vi "AlliGator Clear Parameter & Map Set Rings.vi"(8 "Error In":errorcluster) -> (0 "Error Out":errorcluster)   [LabVIEW 2021, in "AlliGator Parameter Map.lvlib"]
uses:
  AlliGator Parameter Map.lvlib
  AlliGator Parameter Map Control Refnums.ctl
  Globals, Variables, Constants/AlliGator Refnums List.ctl
  GUI/AlliGator GUI.lvlib
panel:
  # "see the License on the block diagram (Ctrl+E or Window:Show Block Diagram)"
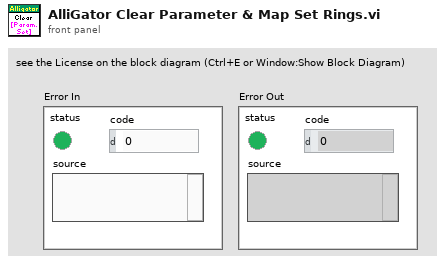
[diagram p1: front panel]
types:
  T1 = typedef "AlliGator GUI.lvlib/AlliGator Refnums List.ctl" = enum16{"---------- AlliGator Control Refnums ----------", "AlliGator Tab Control Refnum", "Dataset Ctrl Refnums", "Image Histogram Ctrl Refnums", "Intensity Time Trace Ctrl Refnums", "Decay Graph Ctrl Refnums", "Decay Statistics Graph Ctrl Refnums", "Phasor Graph Ctrl Refnums", "Phasor Ratio Graph Ctrl Refnums", "Phasor Plot Ctrl Refnums", "Lifetime & Other Parameters Ctrl Refnums", "Decay Fit Parameter Map Ctrl Refnums", "Parameter Map Ctrl Refnums", "Other AlliGator Ctrl Refnums", "---------- AlliGator Menu Refnums ----------", "AlliGator Menu", "---------- AlliGator VI Refnums ----------", "AlliGator Refnum", "AlliGator Settings Refnum", "AlliGator Launcher Refnum", "---------- IO Device ID ----------", "Mouse ID", "Keyboard ID"}
  T2 = typedef "AlliGator Parameter Map.lvlib/AlliGator Parameter Map Control Refnums.ctl" = cluster{"Parameter Map Color Scale":refnum<vi>, "Map Parameter":refnum<vi>, "Max Parameter":refnum<vi>, "Min Parameter":refnum<vi>, "Parameter Map Display":refnum<vi>, "Parameter Map Display Range":refnum<vi>, "Parameter Map Set":refnum<vi>, "Parameter Map X":refnum<vi>, "Parameter Map Y":refnum<vi>, "Parameter Map Value":refnum<vi>}
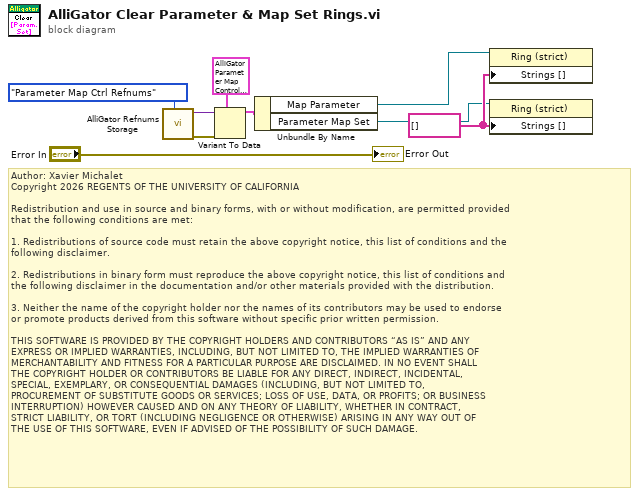
[diagram p0: block diagram]
diagram:
  w8 = string[] [] ("Strings []")
  # "Author: Xavier Michalet\nCopyright 2026 REGENTS OF THE UNIVERSITY OF CALIFORNIA\n\nRedistribution and use in source and binary forms, with or without modification, are permitted provided\nthat the following conditions are met:\n\n1. Redistributions of source code must retain the above copyright notice, this list of conditions and the\nfollowing disclaimer.\n\n2. Redistributions in binary form must reproduce the above copyright notice, this list of conditions and\nthe following disclaimer in the documentation and/or other materials provided with the distribution.\n\n3. Neither the name of the copyright holder nor the names of its contributors may be used to endorse \nor promote products derived from this software without specific prior written permission.\n\nTHIS SOFTWARE IS PROVIDED BY THE COPYRIGHT HOLDERS AND CONTRIBUTORS “AS IS” AND ANY \nEXPRESS OR IMPLIED WARRANTIES, INCLUDING, BUT NOT LIMITED TO, THE IMPLIED WARRANTIES OF\nMERCHANTABILITY AND FITNESS FOR A PARTICULAR PURPOSE ARE DISCLAIMED. IN NO EVENT SHALL\nTHE COPYRIGHT HOLDER OR CONTRIBUTORS BE LIABLE FOR ANY DIRECT, INDIRECT, INCIDENTAL, \nSPECIAL, EXEMPLARY, OR CONSEQUENTIAL DAMAGES (INCLUDING, BUT NOT LIMITED TO, \nPROCUREMENT OF SUBSTITUTE GOODS OR SERVICES; LOSS OF USE, DATA, OR PROFITS; OR BUSINESS\nINTERRUPTION) HOWEVER CAUSED AND ON ANY THEORY OF LIABILITY, WHETHER IN CONTRACT, \nSTRICT LIABILITY, OR TORT (INCLUDING NEGLIGENCE OR OTHERWISE) ARISING IN ANY WAY OUT OF\nTHE USE OF THIS SOFTWARE, EVEN IF ADVISED OF THE POSSIBILITY OF SUCH DAMAGE."
  n1 = call "AlliGator Refnums Storage.vi"("AlliGator Refnum List"=AlliGator_Refnums_List."Parameter Map Ctrl Refnums") -> ("Error Out"=w4:errorcluster, "Data out"=w3:variant)  [unwired: 9 in]
  n2 = Variant To Data(error in=w4, type=T2 {"Parameter Map Color Scale"=refnum, "Map Parameter"=refnum, "Max Parameter"=refnum, "Min Parameter"=refnum, "Parameter Map Display"=refnum, "Parameter Map Display Range"=refnum, "Parameter Map Set"=refnum, "Parameter Map X"=refnum, "Parameter Map Y"=refnum, "Parameter Map Value"=refnum} ("Parameter Map Ctrl Refums"), Variant=w3) -> (data=w9:T2)  [unwired: 1 out]
  n3 = Unbundle By Name(w9) -> ("Map Parameter"=w7:refnum<vi>, "Parameter Map Set"=w6:refnum<vi>)
  n4 = property class="Ring (strict)"(reference=w7, "Strings []"=w8) -> ()  [unwired: 1 in, 2 out]
  n5 = property class="Ring (strict)"(reference=w6, "Strings []"=w8) -> ()  [unwired: 1 in, 2 out]
  "Error Out" <- "Error In"
